vi "subGetDependentLibsFromLinker.vi"(9 "All?":bool, 10 "Owning libs":string[](array[string]), 11 "Paths":path[](array[path])) -> (2 "Dependency files":set{path}(c389), 3 "Dependency libs":T1)   [LabVIEW 2019, in "SolutionBuilder.lvlib" / "SolutionBuilder.lvclass"]
uses:
  SolutionBuilder.lvclass
  NamePathMap.ctl
  SolutionBuilder.lvlib
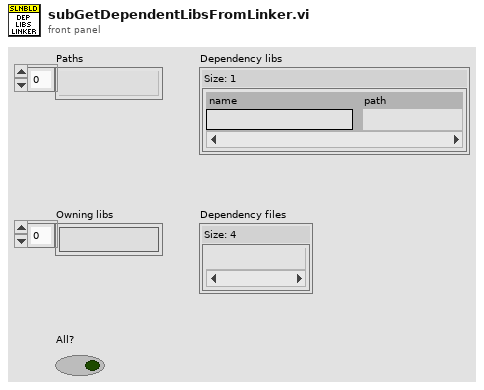
[diagram p1: front panel]
types:
  T1 = typedef "SolutionBuilder.lvlib/SolutionBuilder.lvclass/NamePathMap.ctl" = map{string, path}
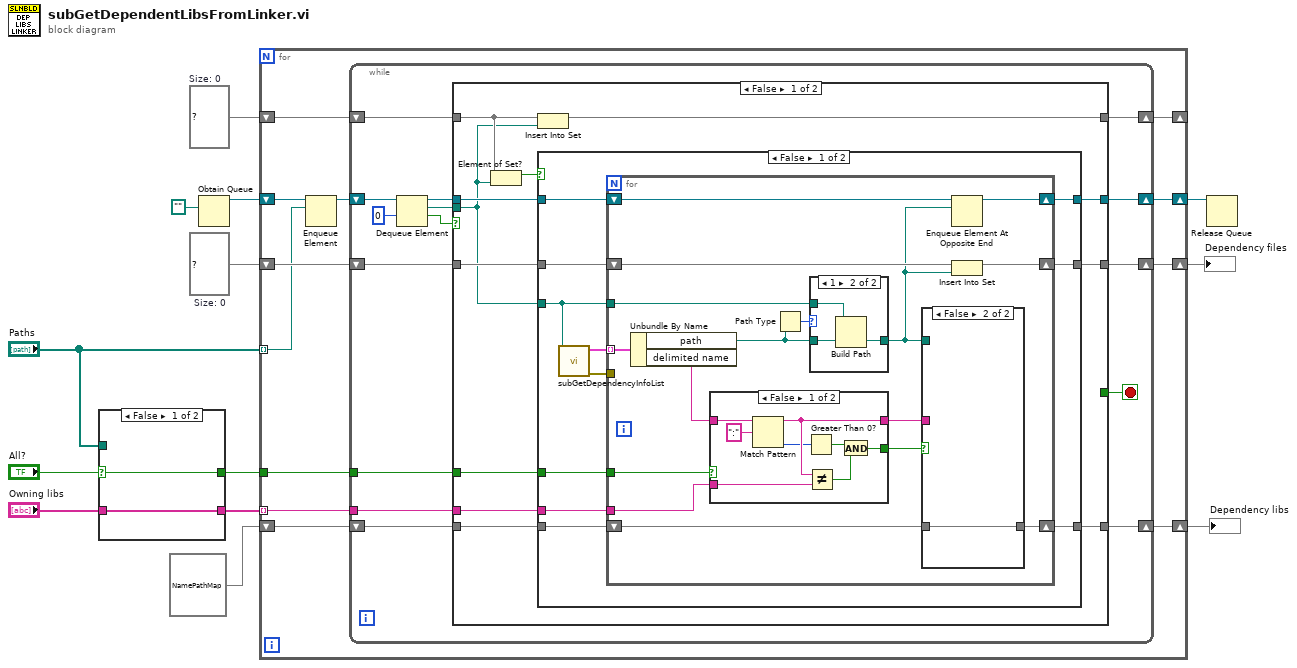
[diagram p0: block diagram]
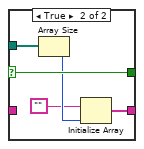
[diagram p2: hidden frame]
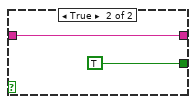
[diagram p3: hidden frame]
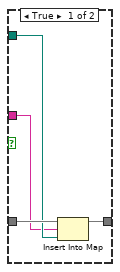
[diagram p5: hidden frame]
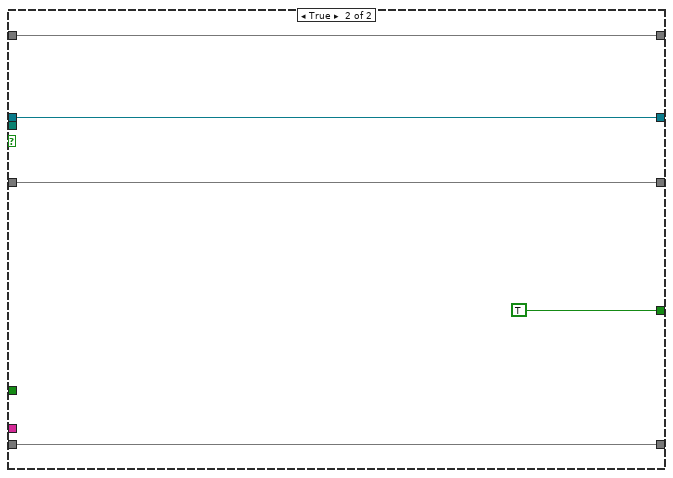
[diagram p7: hidden frame]
diagram:
  w1 = set{path} {}  # Size: 0
  w6 = set{path} {}  # Size: 0
  n1 = case shown="False" "All?" {
    selector: "All?" -> [w14 w19]
    tunnel: "Paths" -> [_ w20]
    tunnel: [w15 w16] -> w9
    tunnel: "Owning libs" -> [w15 _]
    tunnel: [w14 w19] -> w7
    frame False {
    }
    frame True {
      n2 = Array Size(array=w20) -> (size(s)=w18:i32)
      n3 = Initialize Array("", w18) -> (w16:string[])
    }
  }
  n4 = Obtain Queue(element data type=path "") -> (queue out=w3:refnum<queue>)  [unwired: 4 in, 2 out]
  n5 = for {
    tunnel: "Paths" -> [w26] mode=indexing
    shift-right: [w31] -> w13
    shift-left: T1 {} ("Dependency libs") -> [w32]
    tunnel: w9 -> [w30] mode=indexing
    tunnel: w7 -> [w29]
    shift-right: [w27] -> w5
    shift-left: w6 -> [w28]
    shift-right: [w23] -> w2
    shift-left: w3 -> [w24]
    shift-right: [w21] -> _
    shift-left: w1 -> [w22]
    n6 = Enqueue Element(queue=w24, element=w26) -> (queue out=w25:refnum<queue>)  [unwired: 2 in, 2 out]
    n7 = while {
      tunnel: w30 -> [w45]
      tunnel: w29 -> [w44]
      shift-right: [w46] -> w31
      shift-left: w32 -> [w47]
      shift-right: [w42] -> w27
      shift-left: w28 -> [w43]
      shift-right: [w39] -> w23
      shift-left: w25 -> [w41]
      shift-right: [w33] -> w21
      shift-left: w22 -> [w34]
      stop <- w35 stop-if-true
      n8 = Dequeue Element(queue=w41, timeout in ms (-1)=0) -> (queue out=w40:refnum<queue>, element=w37:path, timed out?=w36:bool)  [unwired: 1 in, 1 out]
      n9 = case shown="False" w36 {
        tunnel: w47 -> [w59 w111]
        tunnel: [w58 w111] -> w46
        tunnel: w45 -> [w57 _]
        tunnel: w44 -> [w56 _]
        tunnel: w43 -> [w52 w112]
        tunnel: [w55 w112] -> w42
        tunnel: w40 -> [w54 w113]
        tunnel: [w53 w113] -> w39
        tunnel: w37 -> [w49 _]
        tunnel: [_ TRUE] -> w35
        tunnel: w34 -> [w50 w109]
        tunnel: [w48 w109] -> w33
        frame False {
          n10 = Element of Set?(10:w49, 11:w50) -> (3:w51:bool)
          n11 = Insert Into Set(10:w49, 11:w50) -> (3:w48:set{path})  [unwired: 1 out]
          n12 = case shown="False" w51 {
            tunnel: w59 -> [w70 w106]
            tunnel: [w67 w106] -> w58
            tunnel: w57 -> [w66 _]
            tunnel: w56 -> [w65 _]
            tunnel: [w64 w107] -> w55
            tunnel: w54 -> [w63 w108]
            tunnel: [w62 w108] -> w53
            tunnel: w52 -> [w61 w107]
            tunnel: w49 -> [w60 _]
            frame False {
              n13 = call "subGetDependencyInfoList.vi"("Source path"=w60) -> ("error out"=w68:errorcluster, "Dependencies"=w69:cluster{"path":path, "delimited name":string}[])  [unwired: 9 in]
              n14 = for {
                tunnel: w69 -> [w86] mode=indexing
                shift-right: [w85] -> w67
                shift-left: w70 -> [w84]
                tunnel: w60 -> [w81]
                tunnel: w68 -> [_]
                tunnel: w66 -> [w78]
                tunnel: w65 -> [w76]
                shift-right: [w74] -> w64
                shift-left: w61 -> [w75]
                shift-right: [w72] -> w62
                shift-left: w63 -> [w73]
                n15 = Unbundle By Name(w86) -> ("path"=w82:path, "delimited name"=w80:string)
                n16 = case shown="False" w76 {
                  tunnel: w80 -> [w94 w96]
                  tunnel: [w92 w96] -> w79
                  tunnel: w78 -> [w91 _]
                  tunnel: [w87 TRUE] -> w77
                  frame False {
                    n17 = Match Pattern(string=w94, regular expression=":") -> (before substring=w92:string, offset past match=w90:i32)  [unwired: 1 in, 2 out]
                    n18 = Greater Than 0?(x=w90) -> (x > 0?=w88:bool)
                    n19 = Not Equal?(x=w92, y=w91) -> (x != y?=w89:bool)
                    n20 = And(x=w88, y=w89) -> (x .and. y?=w87:bool)
                  }
                  frame True {
                  }
                }
                n21 = Path Type(1:w82) -> (0:w83:i16)
                n22 = case shown="1" w83 {
                  tunnel: w82 -> [w97 w100]
                  tunnel: w81 -> [_ w99]
                  tunnel: [w97 w98] -> w71
                  frame Default {
                  }
                  frame 1 {
                    n23 = Build Path(base path=w99, name or relative path=w100) -> (appended path=w98:path)
                  }
                }
                n24 = case shown="False" w77 {
                  tunnel: [w102 w105] -> w85
                  tunnel: w84 -> [w104 w105]
                  tunnel: w71 -> [w103 _]
                  tunnel: w79 -> [w101 _]
                  frame True {
                    n25 = Insert Into Map(map in=w104, key=w101, value=w103) -> (map out=w102:T1)  [unwired: 2 out]
                  }
                  frame False {
                  }
                }
                n26 = Enqueue Element At Opposite End(queue=w73, element=w71) -> (queue out=w72:refnum<queue>)  [unwired: 2 in, 2 out]
                n27 = Insert Into Set(10:w71, 11:w75) -> (3:w74:set{path})  [unwired: 1 out]
              }
            }
            frame True {
            }
          }
        }
        frame True {
        }
      }
    }
  }
  "Dependency libs" <- w13
  "Dependency files" <- w5
  n28 = Release Queue(queue=w2) -> ()  [unwired: 2 in, 3 out]
